vi "[ex ce] Data Viewer.vi"() -> ()   [LabVIEW 2021]
doc: "<B>Data Viewer</B>\n\nThe VI displays live and historic data produced by <B>[ex ce] Data acquisition, logging & control.vi</B>.\n\n::: CalcExpress Toolkit :::\nCopyright (c) 2000-2026 Konstantin Shifershteyn. All rights reserved."
panel:
  in  "Mode":enum16{"Live data", "Log Files"}(ring) caption="mode"
  in  "Reversed order":bool=TRUE caption="reversed order"
  out "Message":string
  out "Datalog Folder":path
  in  "Edit Tag List":bool
  out "Table":string[][](table)
  out "Graph":cluster{dbl[], dbl[]}[](graph)
  in  "Update":bool
  out "live data":bool=TRUE
  in  "Timeframe":dbl=120.0 caption="Time Frame" min=60.0 step=30.0 format="%<%H:%M:%S>t"
  in  "Timestamp":timestamp caption="Newest Timestamp" format="%<%X\n%x>T"
  in  "Tag List":i32[](listbox)
  in  "Pause":bool
  in  "Stop":bool
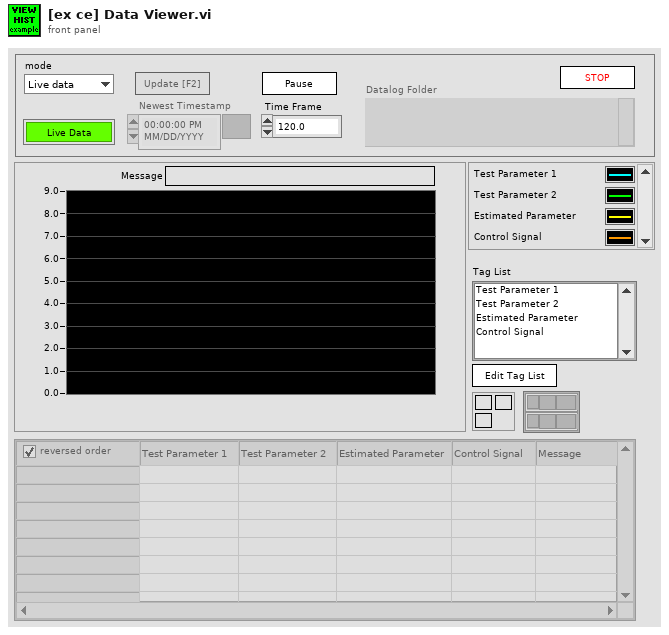
[diagram p1: front panel]
types:
  T1 = cluster{"time stamps out":dbl[], "history data out":dbl[]}
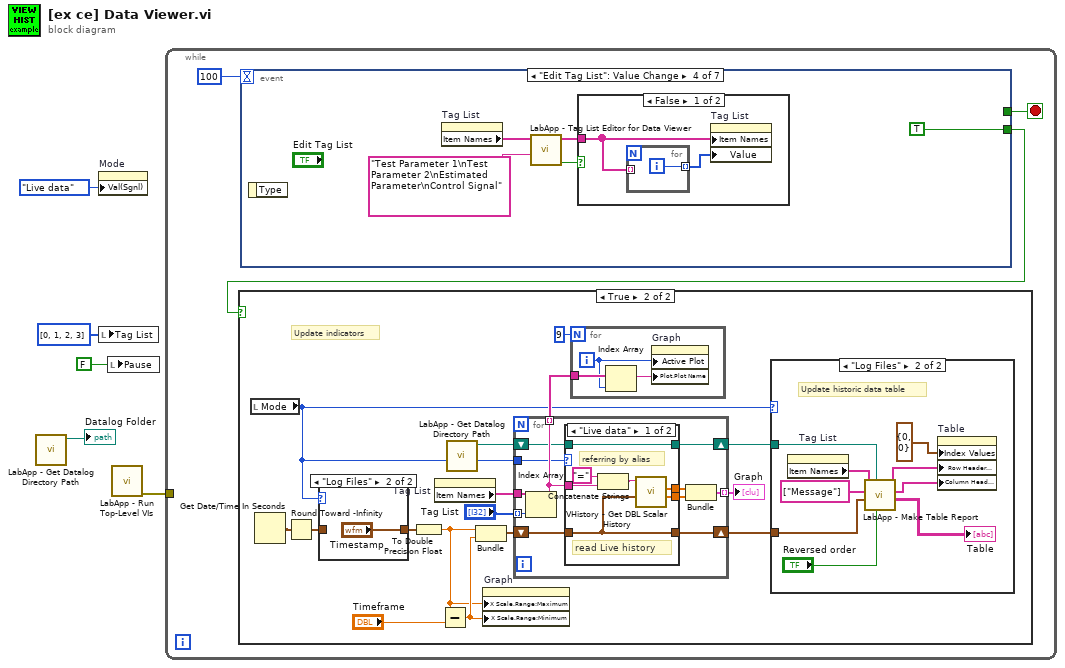
[diagram p0: block diagram]
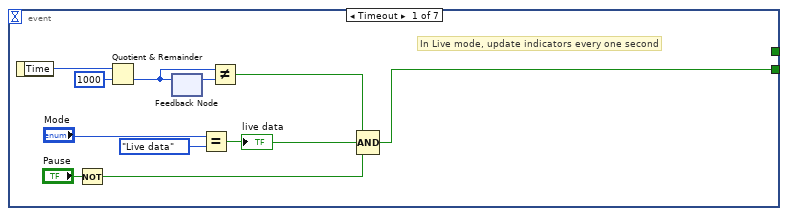
[diagram p2: hidden frame]
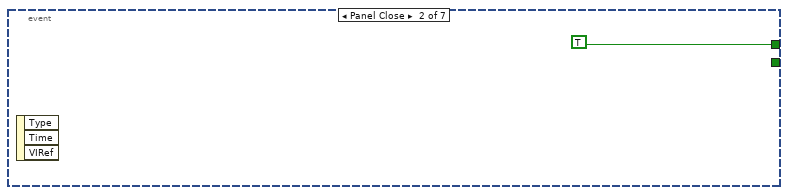
[diagram p3: hidden frame]
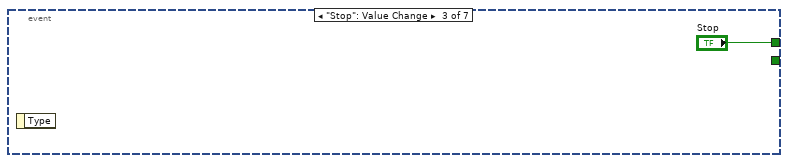
[diagram p4: hidden frame]
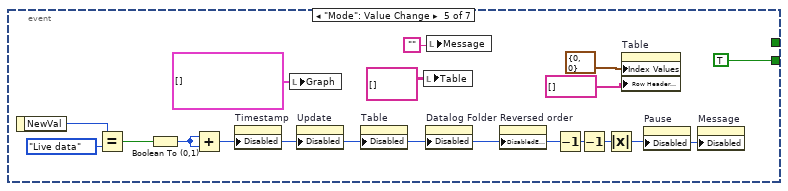
[diagram p6: hidden frame]
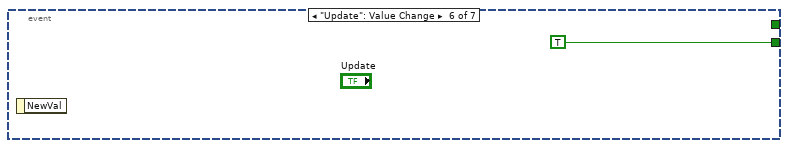
[diagram p7: hidden frame]
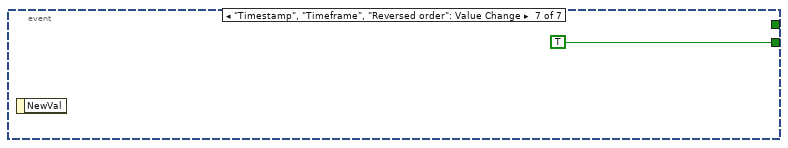
[diagram p8: hidden frame]
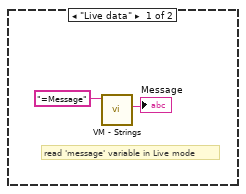
[diagram p10: hidden frame]
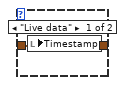
[diagram p11: hidden frame]
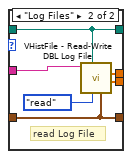
[diagram p12: hidden frame]
diagram:
  n1 = call "LabApp - Get Datalog Directory Path.vi"() -> ("path"=→"Datalog Folder":path)  [unwired: 10 in, 1 out]
  n2 = property on="Mode" class="Enum (strict)"("Val(Sgnl)"=enum16{"Live data", "Log Files"}."Live data" ("Value (Signaling)")) -> ()  [unwired: 2 in, 2 out]
  n3 = local write "Tag List"(i32[] [0, 1, 2, 3] ("Tag List")) -> ()
  n4 = local write "Pause"(FALSE ("pause")) -> ()
  n5 = call "LabApp - Run Top-Level VIs.vi"() -> ("error out"=w3:errorcluster)  [unwired: 9 in]
  n6 = while {
    tunnel: w3 -> [_]
    stop <- w7 stop-if-true
    n7 = event shown="[3] \"Edit Tag List\": Value Change" {
      selector: _ -> [_ _ _ _ _ _ _]
      dyn-events: _ -> [_ _ _ _ _ _ _]
      timeout: 100 -> [_ _ _ _ _ _ _]
      tunnel: [w15 _ _ TRUE TRUE TRUE TRUE] -> w6
      tunnel: [_ TRUE "Stop" _ _ _ _] -> w7
      event Timeout {
        # "In Live mode, update indicators every one second"
        n8 = event-data() -> ("Time"=w13:u32)  [unwired: 1 in]
        n9 = Not(x="Pause") -> (.not. x?=w16:bool)
        n10 = Quotient & Remainder(x=w13, y=u32 1000) -> (floor(x/y)=w10:u32)  [unwired: 1 out]
        n11 = feedback-in #1(w10) -> ()
        n12 = feedback #1() -> (w11:u32)  [unwired: 1 in]
        n13 = Equal?(x="Mode", y=enum16{"Live data", "Log Files"}."Live data") -> (x = y?=w18:bool)
        "live data" <- w18
        n14 = Not Equal?(x=w10, y=w11) -> (x != y?=w9:bool)
        n15 = Compound Arithmetic op=AND(w9, w18, w16) -> (w15:bool)
      }
      event Panel Close {
        n16 = event-data() -> ()  [unwired: 1 in, 3 out]
      }
      event "Stop": Value Change {
        n17 = event-data() -> ()  [unwired: 1 in, 1 out]
      }
      event "Edit Tag List": Value Change {
        n18 = event-data() -> ()  [unwired: 1 in, 1 out]
        n19 = property on="Tag List" class="LstBox (strict)"() -> ("Item Names"=w23:string[])  [unwired: 2 in, 2 out]
        n20 = call "LabApp - Tag List Editor for Data Viewer.vi"("Default"="Test Parameter 1\nTest Parameter 2\nEstimated Parameter\nControl Signal", "Tag List in"=w23) -> ("cancel out"=w24:bool, "Tag List out"=w25:string[])  [unwired: 6 in]
        n21 = case shown="False" w24 {
          tunnel: w25 -> [w28 _]
          frame False {
            n22 = for {
              tunnel: w28 -> [_] mode=indexing
              tunnel: [w29] -> w27 mode=indexing
              i -> [w29]
            }
            n23 = property on="Tag List" class="LstBox (strict)"("Item Names"=w28, "Value"=w27) -> ()  [unwired: 2 in, 2 out]
          }
          frame True {
          }
        }
      }
      event "Mode": Value Change {
        n24 = event-data() -> ("NewVal"=w34:enum16{"Live data", "Log Files"})  [unwired: 1 in]
        n25 = Equal?(x=w34, y=enum16{"Live data", "Log Files"}."Live data") -> (x = y?=w32:bool)
        n26 = Boolean To (0,1)(Boolean=w32) -> (0, 1=w35:i16)
        n27 = Add(x=w35, y=w35) -> (x+y=w30:i16)
        n28 = property on="Timestamp" class="AbsTime (strict)"("Disabled"=w30) -> ()  [unwired: 2 in, 2 out]
        n29 = local write "Graph"(cluster{dbl[], dbl[]}[] [] ("Graph")) -> ()
        n30 = property on="Update" class="Bool"("Disabled"=w30) -> ()  [unwired: 2 in, 2 out]
        n31 = property on="Table" class="Tbl (strict)"("Disabled"=w30) -> ()  [unwired: 2 in, 2 out]
        n32 = local write "Table"(string[][] [] ("report")) -> ()
        n33 = property on="Datalog Folder" class="Path"("Disabled"=w30) -> ()  [unwired: 2 in, 2 out]
        n34 = local write "Message"("") -> ()
        n35 = property on="Reversed order" class="Bool (strict)"("DisabledEnum"=w30) -> ()  [unwired: 2 in, 2 out]
        n36 = Decrement(x=w30) -> (x-1=w38:i16)
        n37 = Decrement(x=w38) -> (x-1=w39:i16)
        n38 = Absolute Value(x=w39) -> (abs(x)=w40:i16)
        n39 = property on="Table" class="Tbl (strict)"("Index Values"=cluster{u32, u32} {0, 0}, "Row Header Strings[]"=string[] [] ("Row Headers[]")) -> ()  [unwired: 2 in, 2 out]
        n40 = property on="Pause" class="Bool (strict)"("Disabled"=w40) -> ()  [unwired: 2 in, 2 out]
        n41 = property on="Message" class="Str"("Disabled"=w40) -> ()  [unwired: 2 in, 2 out]
      }
      event "Update": Value Change {
        n42 = event-data() -> ()  [unwired: 1 in, 1 out]
      }
      event "Timestamp", "Timeframe", "Reversed order": Value Change {
        n43 = event-data() -> ()  [unwired: 1 in, 1 out]
      }
    }
    n44 = case shown="True" w6 {
      frame False {
      }
      frame True {
        # "Update indicators"
        n45 = local read "Mode"() -> (w46:enum16{"Live data", "Log Files"})
        n46 = Get Date/Time In Seconds() -> (seconds since 1Jan1904=w48:timestamp)
        n47 = Round Toward -Infinity(1:w48) -> (0:w47:timestamp)
        n48 = case shown="\"Log Files\"" w46 {
          tunnel: [w73 "Timestamp"] -> w57
          tunnel: w47 -> [w73 _]
          frame "Live data" {
            n49 = local write "Timestamp"(w73) -> ()
          }
          frame "Log Files" {
          }
        }
        n50 = To Double Precision Float(number=w57) -> (double precision float=w50:dbl)
        n51 = property on="Tag List" class="LstBox (strict)"() -> ("Item Names"=w61:string[])  [unwired: 2 in, 2 out]
        n52 = Subtract(x=w50, y="Timeframe") -> (x-y=w56:dbl)
        n53 = call "LabApp - Get Datalog Directory Path.vi"() -> ("path"=w49:path)  [unwired: 10 in, 1 out]
        n54 = Bundle(w50, w56) -> (w53:cluster{dbl, dbl})  [unwired: 1 in]
        n55 = property on="Graph" class="XYGraph (strict)"("X Scale.Range:Maximum"=w50, "X Scale.Range:Minimum"=w56) -> ()  [unwired: 2 in, 2 out]
        n56 = for {
          tunnel: "Tag List" -> [w88] mode=indexing
          tunnel: w61 -> [w87]
          tunnel: [w84] -> w54 mode=indexing
          tunnel: [w83] -> w55 mode=indexing
          tunnel: w46 -> [w82]
          shift-right: [w80] -> w52
          shift-left: w53 -> [w81]
          shift-right: [w78] -> w51
          shift-left: w49 -> [w79]
          n57 = Index Array(array=w87, index=w88) -> (element=w83:string)
          n58 = case shown="\"Live data\"" w82 {
            tunnel: [w93 w101] -> w86
            tunnel: [w92 w100] -> w85
            tunnel: w83 -> [w91 w99]
            tunnel: w81 -> [w90 w98]
            tunnel: w79 -> [w89 w97]
            tunnel: [w90 w98] -> w80
            tunnel: [w89 w97] -> w78
            frame "Live data" {
              # "read Live history"
              # "referring by alias"
              n59 = Concatenate Strings("=", w91) -> (w94:string)
              n60 = call "VHistory - Get DBL Scalar History.vi"("time range (all)"=w90, "name_spec"=w94) -> ("history"=w92:dbl[], "time stamps"=w93:dbl[])  [unwired: 5 in, 3 out]
            }
            frame "Log Files" {
              # "read Log File"
              n61 = call "VHistFile - Read-Write DBL Log File.vi"("time range to read"=w98, "operation"=enum16{"nop", "read", "write", "retrieve"}."read", "log directory"=w97, "file tag"=w99) -> ("history data out"=w100:dbl[], "time stamps out"=w101:dbl[])  [unwired: 5 in, 1 out]
            }
          }
          n62 = Bundle("time stamps out"=w86, "history data out"=w85) -> (w84:T1)  [unwired: 1 in]
        }
        "Graph" <- w54
        n63 = for {
          N: 9 -> [_]
          tunnel: w55 -> [w77]
          i -> [w76]
          n64 = Index Array(array=w77, index=w76) -> (element=w75:string)
          n65 = property on="Graph" class="XYGraph (strict)"("Active Plot"=w76, "Plot.Plot Name"=w75) -> ()  [unwired: 2 in, 2 out]
        }
        n66 = case shown="\"Log Files\"" w46 {
          tunnel: w52 -> [_ w70]
          tunnel: w51 -> [_ w69]
          frame "Live data" {
            # "read 'message' variable in Live mode"
            n67 = call "VM - Strings.vi"("name_spec"="=Message") -> ("value out"=→"Message":string)  [unwired: 5 in, 5 out]
          }
          frame "Log Files" {
            # "Update historic data table"
            n68 = property on="Tag List" class="LstBox (strict)"() -> ("Item Names"=w71:string[])  [unwired: 2 in, 2 out]
            n69 = call "LabApp - Make Table Report.vi"("reverse order (F)"="Reversed order", "log directory"=w69, "time range"=w70, "Str Tags"=string[] ["Message"], "Num Tags"=w71) -> ("Report Data"=→"Table":string[][], "Column Headers (Tags)"=w67:string[], "Row Headers (timestamps)"=w66:string[])  [unwired: 4 in]
            n70 = property on="Table" class="Tbl (strict)"("Index Values"=cluster{u32, u32} {0, 0}, "Row Header Strings[]"=w66, "Column Header Strings[]"=w67) -> ()  [unwired: 2 in, 2 out]
          }
        }
      }
    }
  }
